vi "get information display strings.vi"(8 "error in":errorcluster, 11 "NISE_CEF_serializable node in":refnum<class "NISE_CEF_serializable node.lvclass">) -> (0 "error out":errorcluster, 1 "Data":string[](array[string]), 2 "Labels":string[](array[string]), 3 "NISE_CEF_serializable node out":refnum<class "NISE_CEF_serializable node.lvclass">)   [LabVIEW 2014, in "NISE_CEF_serializable node.lvclass"]
uses:
  NISE_CEF_serializable node.lvclass
  serializable configuration/NISE_CEF_serializable configuration.lvclass/NISE_CEF_serializable configuration.ctl
  <vilib>/Utility/LVClass/Get LV Class Name.vi
  error generator/NISE_error generator.vi
  serializable configuration/NISE_CEF_serializable configuration.lvclass
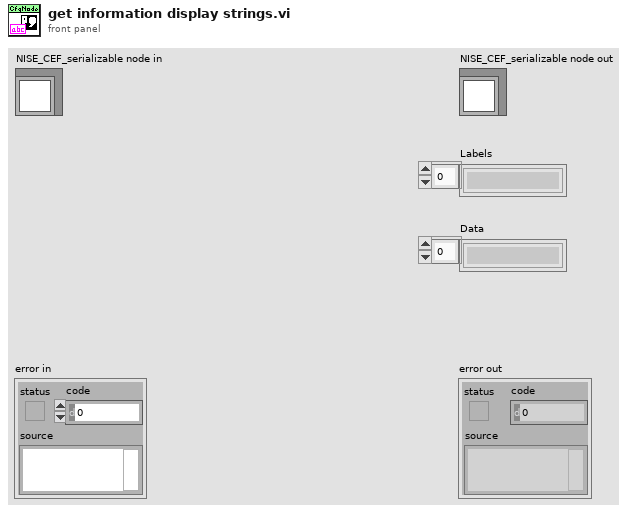
[diagram p1: front panel]
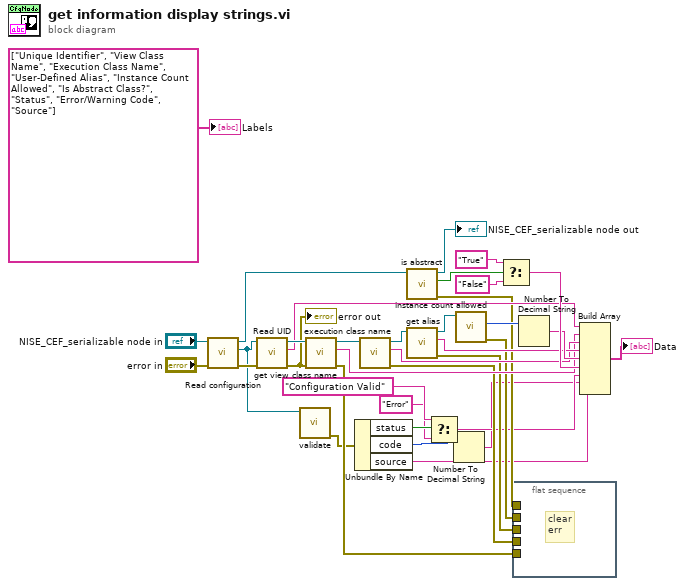
[diagram p0: block diagram]
diagram:
  n1 = call-dynamic "Read configuration.vi"("error in"="error in", "NISE_CEF_serializable node in"="NISE_CEF_serializable node in") -> ("error out"=w28:errorcluster, "configuration"=w9:refnum<class "NISE_CEF_serializable configuration.lvclass">, "NISE_CEF_serializable node out"=w33:refnum<class "NISE_CEF_serializable node.lvclass">)  [unwired: 7 in]
  n2 = call "Read UID.vi"("error in"=w28, "configuration in"=w9) -> ("error out"=w15:errorcluster, "instance id"=w16:string, "configuration out"=w32:refnum<class "NISE_CEF_serializable configuration.lvclass">)  [unwired: 7 in]
  "error out" <- w15
  n3 = call-dynamic "validate.vi"("configuration in"=w9) -> ("error out"=w8:errorcluster)  [unwired: 9 in, 1 out]
  n4 = call "get view class name.vi"("error in"=w15, "configuration in"=w32) -> ("error out"=w14:errorcluster, "view class"=w17:string, "configuration out"=w31:refnum<class "NISE_CEF_serializable configuration.lvclass">)  [unwired: 7 in]
  n5 = Unbundle By Name(w8) -> ("status"=w7:bool, "code"=w2:i32, "source"=w3:string)
  n6 = call-dynamic "execution class name.vi"("configuration in"=w31) -> ("error out"=w13:errorcluster, "execution class"=w18:string, "configuration out"=w30:refnum<class "NISE_CEF_serializable configuration.lvclass">)  [unwired: 8 in]
  n7 = call-dynamic "is abstract.vi"("NISE_CEF_serializable node in"=w33) -> ("error out"=w10:errorcluster, "abstract"=w26:bool, "NISE_CEF_serializable node out"=→"NISE_CEF_serializable node out":refnum<class "NISE_CEF_serializable node.lvclass">)  [unwired: 8 in]
  n8 = call "get alias.vi"("configuration in"=w30) -> ("error out"=w12:errorcluster, "alias"=w19:string, "configuration out"=w29:refnum<class "NISE_CEF_serializable configuration.lvclass">)  [unwired: 8 in]
  n9 = Select(t="Configuration Valid", s=w7, f="Error") -> (s? t:f=w4:string)
  n10 = Number To Decimal String(number=w2) -> (decimal integer string=w1:string)  [unwired: 1 in]
  n11 = call-dynamic "instance count allowed.vi"("configuration in"=w29) -> ("error out"=w11:errorcluster, "instances allowed"=w21:i32)  [unwired: 8 in, 1 out]
  n12 = Select(t="True", s=w26, f="False") -> (s? t:f=w23:string)
  n13 = flat-sequence {
    tunnel: w14 -> [_]
    tunnel: w13 -> [_]
    tunnel: w12 -> [_]
    tunnel: w11 -> [_]
    tunnel: w10 -> [_]
    frame #0 {
      # "clear\nerr"
    }
  }
  n14 = Number To Decimal String(number=w21) -> (decimal integer string=w20:string)  [unwired: 1 in]
  n15 = Build Array(w16, w17, w18, w19, w20, w23, w4, w1, w3) -> (→"Data":string[])
  "Labels" <- string[] ["Unique Identifier", "View Class Name", "Execution Class Name", "User-Defined Alias", "Instance Count Allowed", "Is Abstract Class?", "Status", "Error/Warning Code", "Source"] ("Labels")
